vi "FX_Open.vi"(4 "error in (no error)":errorcluster, 8 "COM Port":refnum<visa-resource-name>, 9 "Port":u16, 10 "Host":string, 11 "Transport":T1(ring)) -> (2 "error out":errorcluster, 3 "PLC Conn":refnum<visa-resource-name>)   [LabVIEW 2018]
doc: "Use this template to build a VI to use as a subVI."
panel:
  # "說明：開通訊。TCP 給模擬器，RS-422、USB 走 COM 埠\n，固定 9600、7 位、偶校驗、1 停止位。送 ENQ 收到 AC\nK 才算連上。"
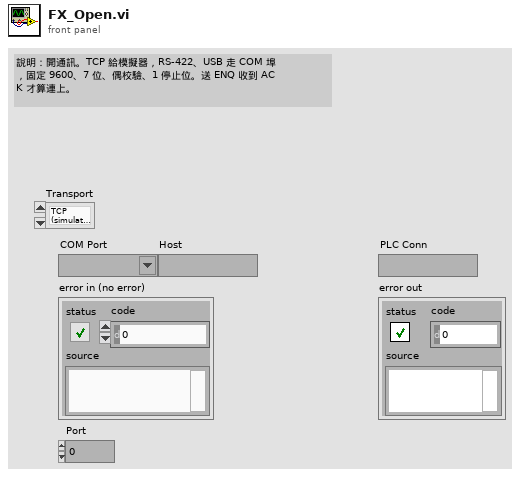
[diagram p1: front panel]
types:
  T1 = enum16{"TCP (simulator)", "RS-422 (COM)", "USB (COM)"}
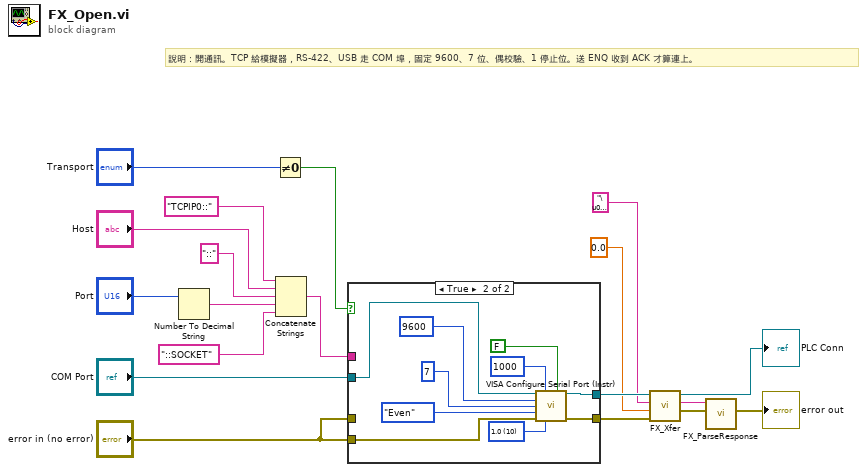
[diagram p0: block diagram]
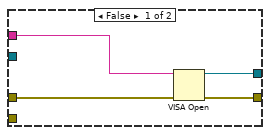
[diagram p2: hidden frame]
diagram:
  # "說明：開通訊。TCP 給模擬器，RS-422、USB 走 COM 埠，固定 9600、7 位、偶校驗、1 停止位。送 ENQ 收到 ACK 才算連上。"
  n1 = Number To Decimal String(number="Port") -> (decimal integer string=w14:string)  [unwired: 1 in]
  n2 = Not Equal To 0?(x="Transport") -> (x != 0?=w12:bool)
  n3 = Concatenate Strings("TCPIP0::", "Host", "::", w14, "::SOCKET") -> (w11:string)
  n4 = case shown="True" w12 {
    tunnel: w11 -> [w23 _]
    tunnel: "error in (no error)" -> [w22 _]
    tunnel: "COM Port" -> [_ w33]
    tunnel: "error in (no error)" -> [_ w32]
    tunnel: [w21 w25] -> w8
    tunnel: [w20 w24] -> w7
    frame False {
      n5 = VISA Open(error in (no error)=w22, VISA resource name=w23) -> (VISA resource name=w21:refnum<visa-resource-name>, error out=w20:errorcluster)  [unwired: 3 in]
    }
    frame True {
      w28 = u16 10 items=["1.0"=10, "1.5"=15, "2.0"=20] ("stop bits (10: 1 bit)")
      n6 = call <vilib>:"VISA Configure Serial Port (Instr).vi"("VISA resource name"=w33, "timeout (10sec)"=u32 1000, "Enable Termination\nChar (T)"=FALSE, "baud rate (9600)"=u32 9600, "data bits (8)"=u16 7, "parity (0:none)"=enum16{"None", "Odd", "Even", "Mark", "Space"}."Even", "error in (no error)"=w32, "stop bits (10: 1 bit)"=w28) -> ("VISA resource name out"=w25:refnum<visa-resource-name>, "error out"=w24:errorcluster)  [unwired: 6 in]
    }
  }
  n7 = call "FX_Xfer.vi"("error in (no error)"=w7, "Data Chars"=0.0, "TX"="\u0005", "PLC Conn"=w8) -> ("error out"=w3:errorcluster, "RX"=w4:string, "PLC Conn out"=→"PLC Conn":refnum<visa-resource-name>)  [unwired: 5 in]
  n8 = call "FX_ParseResponse.vi"("error in (no error)"=w3, "RX"=w4) -> ("error out"=→"error out":errorcluster)  [unwired: 8 in, 1 out]
